vi "modbus Profibus.vi"() -> (4 "OffCoil":T4, 6 "On Coil":T3, 8 "cluster":T1, 10 "Temp":T2)   [LabVIEW 2025]
uses:
  <vilib>/Modbus/master/Modbus Master.lvclass
  <vilib>/Analysis/NI_AALBase.lvlib
  <vilib>/Analysis/baseanly.llb/Mean (DBL).vi
  <vilib>/Modbus/master/Create Master Instance (TCP).vi
panel:
  in  "Boolean":bool
  out "TREES AVG array":dbl[](array[numeric])
  out "OD_Right side AVG distributed":dbl format="%0.2f"
  out "ON_Coil AVG distributed":dbl format="%0.2f"
  out "OFF_Coil AVG distributed":dbl format="%0.2f"
  out "AMB RIGHT":dbl[](array[numeric])
  out "ON-COIL 2":dbl[](array[numeric])
  out "OFF-COIL 2":dbl[](array[numeric])
  out "error out":errorcluster
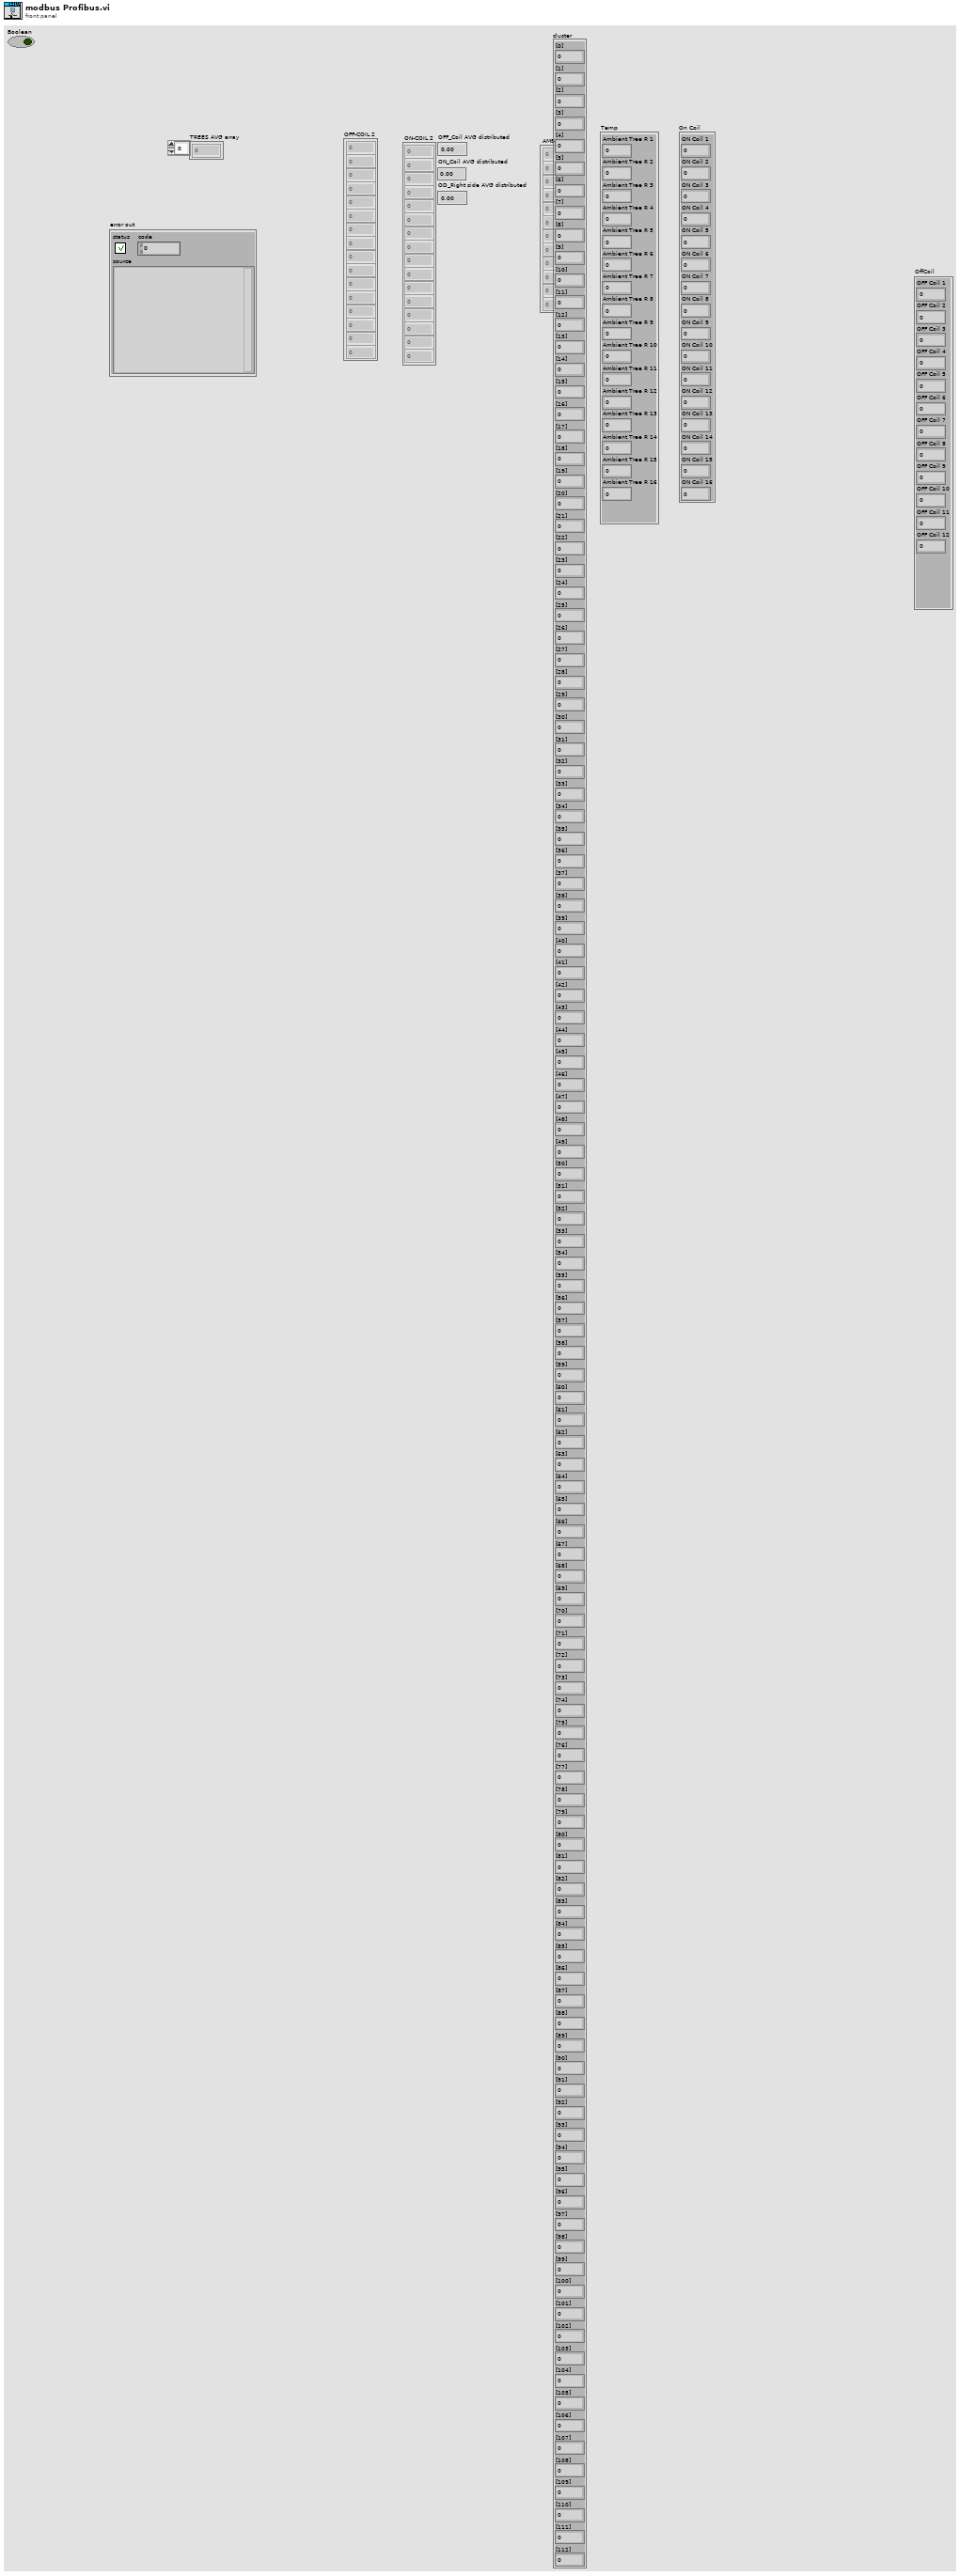
[diagram p1: front panel]
types:
  T1 = cluster{"[0]":dbl, "[1]":dbl, "[2]":dbl, "[3]":dbl, "[4]":dbl, "[5]":dbl, "[6]":dbl, "[7]":dbl, "[8]":dbl, "[9]":dbl, "[10]":dbl, "[11]":dbl, "[12]":dbl, "[13]":dbl, "[14]":dbl, "[15]":dbl, "[16]":dbl, "[17]":dbl, "[18]":dbl, "[19]":dbl, "[20]":dbl, "[21]":dbl, "[22]":dbl, "[23]":dbl, "[24]":dbl, "[25]":dbl, "[26]":dbl, "[27]":dbl, "[28]":dbl, "[29]":dbl, "[30]":dbl, "[31]":dbl, "[32]":dbl, "[33]":dbl, "[34]":dbl, "[35]":dbl, "[36]":dbl, "[37]":dbl, "[38]":dbl, "[39]":dbl, "[40]":dbl, "[41]":dbl, "[42]":dbl, "[43]":dbl, "[44]":dbl, "[45]":dbl, "[46]":dbl, "[47]":dbl, "[48]":dbl, "[49]":dbl, "[50]":dbl, "[51]":dbl, "[52]":dbl, "[53]":dbl, "[54]":dbl, "[55]":dbl, "[56]":dbl, "[57]":dbl, "[58]":dbl, "[59]":dbl, "[60]":dbl, "[61]":dbl, "[62]":dbl, "[63]":dbl, "[64]":dbl, "[65]":dbl, "[66]":dbl, "[67]":dbl, "[68]":dbl, "[69]":dbl, "[70]":dbl, "[71]":dbl, "[72]":dbl, "[73]":dbl, "[74]":dbl, "[75]":dbl, "[76]":dbl, "[77]":dbl, "[78]":dbl, "[79]":dbl, "[80]":dbl, "[81]":dbl, "[82]":dbl, "[83]":dbl, "[84]":dbl, "[85]":dbl, "[86]":dbl, "[87]":dbl, "[88]":dbl, "[89]":dbl, "[90]":dbl, "[91]":dbl, "[92]":dbl, "[93]":dbl, "[94]":dbl, "[95]":dbl, "[96]":dbl, "[97]":dbl, "[98]":dbl, "[99]":dbl, "[100]":dbl, "[101]":dbl, "[102]":dbl, "[103]":dbl, "[104]":dbl, "[105]":dbl, "[106]":dbl, "[107]":dbl, "[108]":dbl, "[109]":dbl, "[110]":dbl, "[111]":dbl, "[112]":dbl}
  T2 = cluster{"Ambient Tree R 1":dbl, "Ambient Tree R 2":dbl, "Ambient Tree R 3":dbl, "Ambient Tree R 4":dbl, "Ambient Tree R 5":dbl, "Ambient Tree R 6":dbl, "Ambient Tree R 7":dbl, "Ambient Tree R 8":dbl, "Ambient Tree R 9":dbl, "Ambient Tree R 10":dbl, "Ambient Tree R 11":dbl, "Ambient Tree R 12":dbl, "Ambient Tree R 13":dbl, "Ambient Tree R 14":dbl, "Ambient Tree R 15":dbl, "Ambient Tree R 16":dbl}
  T3 = cluster{"ON Coil 1":dbl, "ON Coil 2":dbl, "ON Coil 3":dbl, "ON Coil 4":dbl, "ON Coil 5":dbl, "ON Coil 6":dbl, "ON Coil 7":dbl, "ON Coil 8":dbl, "ON Coil 9":dbl, "ON Coil 10":dbl, "ON Coil 11":dbl, "ON Coil 12":dbl, "ON Coil 13":dbl, "ON Coil 14":dbl, "ON Coil 15":dbl, "ON Coil 16":dbl}
  T4 = cluster{"OFF Coil 1":dbl, "OFF Coil 2":dbl, "OFF Coil 3":dbl, "OFF Coil 4":dbl, "OFF Coil 5":dbl, "OFF Coil 6":dbl, "OFF Coil 7":dbl, "OFF Coil 8":dbl, "OFF Coil 9":dbl, "OFF Coil 10":dbl, "OFF Coil 11":dbl, "OFF Coil 12":dbl}
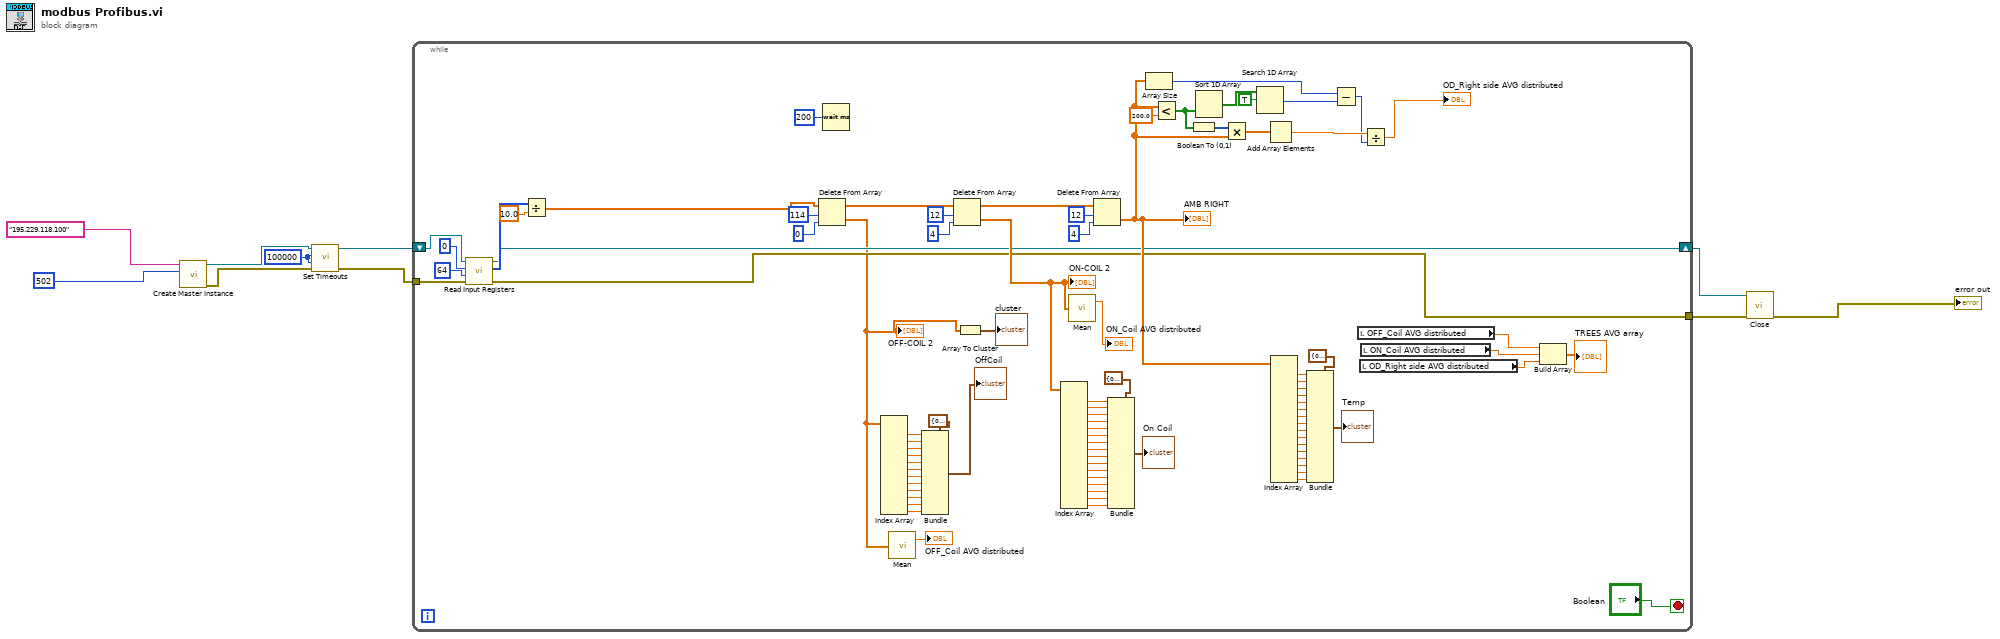
[diagram p0: block diagram]
diagram:
  w4 = 100000 ("read operation timeout (ms)")
  n1 = call-poly <vilib>:"Create Master Instance.vi"("port (502)"=u16 502, "address"="195.229.118.100") -> ("error out"=w5:errorcluster, "TCP master instance"=w6:refnum<class "Modbus Master.lvclass">)  [unwired: 8 in]
  n2 = call <vilib>:"Set Timeouts.vi"("error in (no error)"=w5, "write operation timeout (ms)"=w4, "read operation timeout (ms)"=w4, "Modbus master in"=w6) -> ("error out"=w10:errorcluster, "Modbus master out"=w9:refnum<class "Modbus Master.lvclass">)  [unwired: 6 in]
  n3 = while {
    tunnel: w10 -> [w22]
    tunnel: [w15] -> w2
    shift-right: [w14] -> w1
    shift-left: w9 -> [w21]
    stop <- "Boolean" stop-if-true
    n4 = call-dynamic "Read Input Registers.vi"("error in (no error)"=w22, "number of input registers"=u16 64, "starting address"=u16 0, "Modbus master in"=w21) -> ("error out"=w15:errorcluster, "register values"=w19:u16[], "Modbus master out"=w14:refnum<class "Modbus Master.lvclass">)  [unwired: 5 in]
    n5 = Divide(x=w19, y=10.0) -> (x/y=w23:dbl[])
    n6 = Delete From Array(array=w23, length=114, index=0) -> (deleted portion=w12:dbl[], array with subset deleted=w96:dbl[])
    "OFF-COIL 2" <- w12
    n7 = Wait (ms)(milliseconds to wait=u32 200) -> ()  [unwired: 1 out]
    n8 = Index Array(array=w12) -> (element #1=w89:dbl, element #2=w88:dbl, element #3=w87:dbl, element #4=w86:dbl, element #5=w85:dbl, element #6=w84:dbl, element #7=w83:dbl, element #8=w82:dbl, element #9=w81:dbl, element #10=w80:dbl, element #11=w79:dbl, element #12=w78:dbl)  [unwired: 12 in]
    n9 = call-poly <vilib>:"Mean.vi"("X"=w12) -> ("mean"=→"OFF_Coil AVG distributed":dbl)  [unwired: 1 out]
    n10 = Bundle(cluster=T4 {"OFF Coil 1"=0.0, "OFF Coil 2"=0.0, "OFF Coil 3"=0.0, "OFF Coil 4"=0.0, "OFF Coil 5"=0.0, "OFF Coil 6"=0.0, "OFF Coil 7"=0.0, "OFF Coil 8"=0.0, "OFF Coil 9"=0.0, "OFF Coil 10"=0.0, "OFF Coil 11"=0.0, "OFF Coil 12"=0.0}, "OFF Coil 1"=w89, "OFF Coil 2"=w88, "OFF Coil 3"=w87, "OFF Coil 4"=w86, "OFF Coil 5"=w85, "OFF Coil 6"=w84, "OFF Coil 7"=w83, "OFF Coil 8"=w82, "OFF Coil 9"=w81, "OFF Coil 10"=w80, "OFF Coil 11"=w79, "OFF Coil 12"=w78) -> (→"OffCoil":T4)
    n11 = Delete From Array(array=w96, length=12, index=4) -> (deleted portion=w76:dbl[], array with subset deleted=w93:dbl[])
    "ON-COIL 2" <- w76
    n12 = Array To Cluster(array=w12) -> (cluster=→"cluster":T1)
    n13 = Index Array(array=w76) -> (element #1=w74:dbl, element #2=w73:dbl, element #3=w72:dbl, element #4=w71:dbl, element #5=w70:dbl, element #6=w69:dbl, element #7=w68:dbl, element #8=w67:dbl, element #9=w66:dbl, element #10=w65:dbl, element #11=w64:dbl, element #12=w63:dbl, element #13=w62:dbl, element #14=w61:dbl, element #15=w60:dbl, element #16=w59:dbl)  [unwired: 16 in]
    n14 = call-poly <vilib>:"Mean.vi"("X"=w76) -> ("mean"=→"ON_Coil AVG distributed":dbl)  [unwired: 1 out]
    n15 = Delete From Array(array=w93, length=12, index=4) -> (deleted portion=w30:dbl[])  [unwired: 1 out]
    "AMB RIGHT" <- w30
    n16 = Bundle(cluster=T3 {"ON Coil 1"=0.0, "ON Coil 2"=0.0, "ON Coil 3"=0.0, "ON Coil 4"=0.0, "ON Coil 5"=0.0, "ON Coil 6"=0.0, "ON Coil 7"=0.0, "ON Coil 8"=0.0, "ON Coil 9"=0.0, "ON Coil 10"=0.0, "ON Coil 11"=0.0, "ON Coil 12"=0.0, "ON Coil 13"=0.0, "ON Coil 14"=0.0, "ON Coil 15"=0.0, "ON Coil 16"=0.0}, "ON Coil 1"=w74, "ON Coil 2"=w73, "ON Coil 3"=w72, "ON Coil 4"=w71, "ON Coil 5"=w70, "ON Coil 6"=w69, "ON Coil 7"=w68, "ON Coil 8"=w67, "ON Coil 9"=w66, "ON Coil 10"=w65, "ON Coil 11"=w64, "ON Coil 12"=w63, "ON Coil 13"=w62, "ON Coil 14"=w61, "ON Coil 15"=w60, "ON Coil 16"=w59) -> (→"On Coil":T3)
    n17 = Array Size(array=w30) -> (size(s)=w32:i32)
    n18 = Less?(x=w30, y=200.0) -> (x < y?=w29:bool[])
    n19 = Boolean To (0,1)(Boolean=w29) -> (0, 1=w28:i16[])
    n20 = Sort 1D Array(array=w29) -> (sorted array=w34:bool[])
    n21 = Multiply(x=w28, y=w30) -> (x*y=w27:dbl[])
    n22 = Search 1D Array(1D array=w34, element=TRUE) -> (index of element=w31:i32)  [unwired: 1 in]
    n23 = Add Array Elements(numeric array=w27) -> (sum=w26:dbl)
    n24 = Index Array(array=w30) -> (element #1=w56:dbl, element #2=w55:dbl, element #3=w54:dbl, element #4=w53:dbl, element #5=w52:dbl, element #6=w51:dbl, element #7=w50:dbl, element #8=w49:dbl, element #9=w48:dbl, element #10=w47:dbl, element #11=w46:dbl, element #12=w45:dbl, element #13=w44:dbl, element #14=w43:dbl, element #15=w42:dbl, element #16=w41:dbl)  [unwired: 16 in]
    n25 = Bundle(cluster=T2 {"Ambient Tree R 1"=0.0, "Ambient Tree R 2"=0.0, "Ambient Tree R 3"=0.0, "Ambient Tree R 4"=0.0, "Ambient Tree R 5"=0.0, "Ambient Tree R 6"=0.0, "Ambient Tree R 7"=0.0, "Ambient Tree R 8"=0.0, "Ambient Tree R 9"=0.0, "Ambient Tree R 10"=0.0, "Ambient Tree R 11"=0.0, "Ambient Tree R 12"=0.0, "Ambient Tree R 13"=0.0, "Ambient Tree R 14"=0.0, "Ambient Tree R 15"=0.0, "Ambient Tree R 16"=0.0}, "Ambient Tree R 1"=w56, "Ambient Tree R 2"=w55, "Ambient Tree R 3"=w54, "Ambient Tree R 4"=w53, "Ambient Tree R 5"=w52, "Ambient Tree R 6"=w51, "Ambient Tree R 7"=w50, "Ambient Tree R 8"=w49, "Ambient Tree R 9"=w48, "Ambient Tree R 10"=w47, "Ambient Tree R 11"=w46, "Ambient Tree R 12"=w45, "Ambient Tree R 13"=w44, "Ambient Tree R 14"=w43, "Ambient Tree R 15"=w42, "Ambient Tree R 16"=w41) -> (→"Temp":T2)
    n26 = Subtract(x=w32, y=w31) -> (x-y=w25:i32)
    n27 = local read "OFF_Coil AVG distributed"() -> (w39:dbl)
    n28 = local read "OD_Right side AVG distributed"() -> (w37:dbl)
    n29 = local read "ON_Coil AVG distributed"() -> (w38:dbl)
    n30 = Divide(x=w26, y=w25) -> (x/y=→"OD_Right side AVG distributed":dbl)
    n31 = Build Array(w39, w38, w37) -> (→"TREES AVG array":dbl[])
  }
  n32 = call-dynamic "Close.vi"("error in (no error)"=w2, "Modbus master in"=w1) -> ("error out"=→"error out":errorcluster)  [unwired: 9 in]
